vi "Update measured value.vi"(8 "error in (no error) 2":errorcluster, 9 "MEASURED":string, 10 "HI SET":string, 11 "LO SET":string) -> (0 "error in (no error) 3":errorcluster, 1 "MEASURED":string, 2 "HI SET":string, 3 "LO SET":string)   [LabVIEW 2021]
uses:
  Control/Ini.ctl
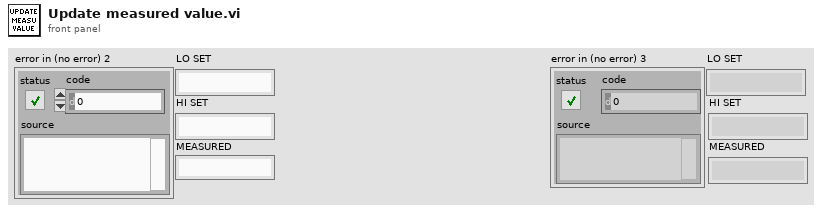
[diagram p1: front panel]
types:
  T1 = typedef "Ini.ctl" = enum16{"Write", "Read"}
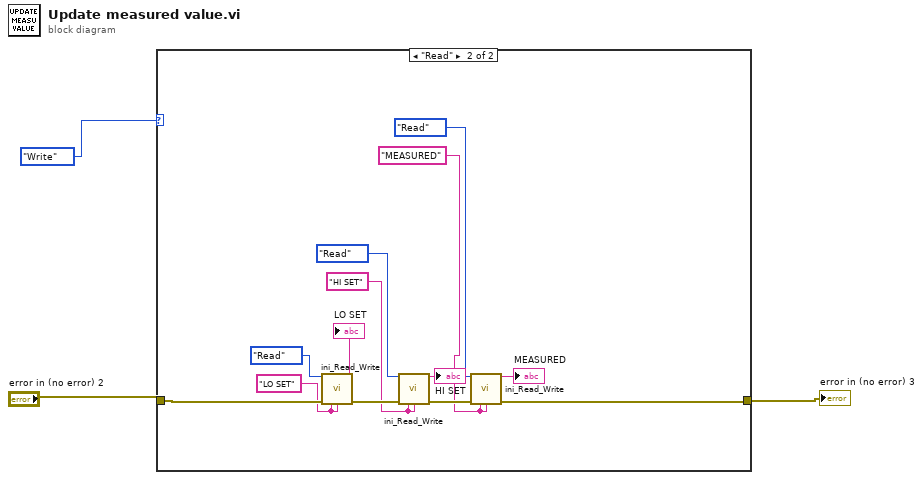
[diagram p0: block diagram]
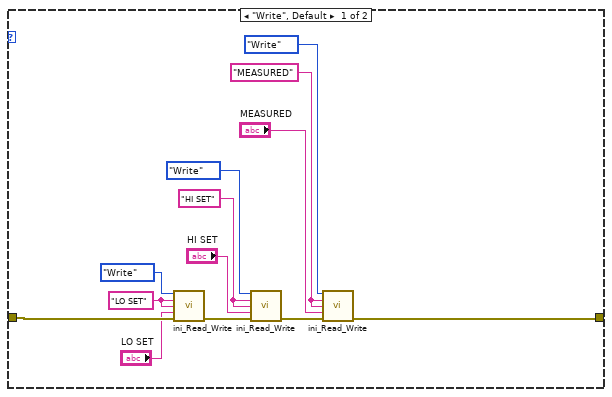
[diagram p2: hidden frame]
diagram:
  n1 = case shown="\"Read\"" Ini."Write" {
    tunnel: [w8 w24] -> w2
    tunnel: "error in (no error) 2" -> [w7 w23]
    frame "Write", Default {
      w11 = "MEASURED" ("Write Section")
      w13 = "HI SET" ("Write Section")
      w15 = "LO SET" ("Write Section")
      n2 = call "ini_Read_Write.vi"(0:Ini."Write", "Write Section"=w15, "Write key"=w15, "Write"="LO SET", "error in (no error) 2"=w7) -> ("error in (no error) 3"=w10:errorcluster)  [unwired: 9 in, 1 out]
      n3 = call "ini_Read_Write.vi"(0:Ini."Write", "Write Section"=w13, "Write key"=w13, "Write"="HI SET", "error in (no error) 2"=w10) -> ("error in (no error) 3"=w9:errorcluster)  [unwired: 9 in, 1 out]
      n4 = call "ini_Read_Write.vi"(0:Ini."Write", "Write Section"=w11, "Write key"=w11, "Write"="MEASURED", "error in (no error) 2"=w9) -> ("error in (no error) 3"=w8:errorcluster)  [unwired: 9 in, 1 out]
    }
    frame "Read" {
      w20 = "MEASURED" ("Write Section")
      w21 = "HI SET" ("Write Section")
      w22 = "LO SET" ("Write Section")
      n5 = call "ini_Read_Write.vi"(0:Ini."Read", "error in (no error) 2"=w23, "Read Section"=w22, "Read Key"=w22) -> ("value"=→"LO SET":string, "error in (no error) 3"=w26:errorcluster)  [unwired: 10 in]
      n6 = call "ini_Read_Write.vi"(0:Ini."Read", "error in (no error) 2"=w26, "Read Section"=w21, "Read Key"=w21) -> ("value"=→"HI SET":string, "error in (no error) 3"=w25:errorcluster)  [unwired: 10 in]
      n7 = call "ini_Read_Write.vi"(0:Ini."Read", "error in (no error) 2"=w25, "Read Section"=w20, "Read Key"=w20) -> ("value"=→"MEASURED":string, "error in (no error) 3"=w24:errorcluster)  [unwired: 10 in]
    }
  }
  "error in (no error) 3" <- w2
